vi "Transport_Receive_Command.vi"(8 "error in (no error)":errorcluster={"status"=FALSE, "code"=0, "source"="\"\""}, 10 "shutdown token":string, 11 "Transport ref":string) -> (0 "error out":errorcluster={"status"=FALSE, "code"=0, "source"="\"\""}, 2 "status ok":bool, 3 "RuntimeMessage":string)   [LabVIEW 2026]
doc: "INTENT: Consume incoming target requests. LOGIC: Read with bounded timeout; decode and validate envelope; reject malformed messages."
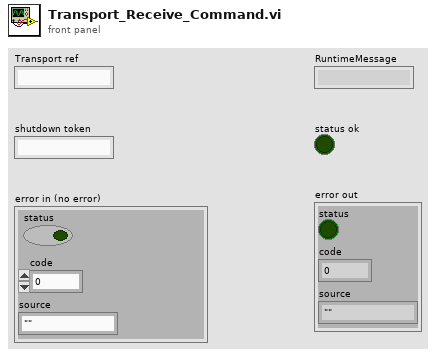
[diagram p1: front panel]
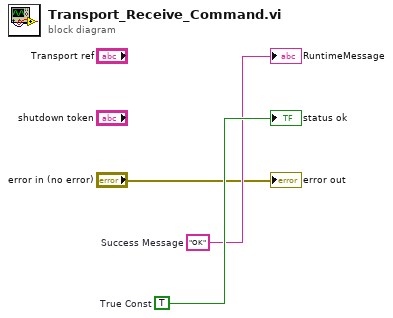
[diagram p0: block diagram]
diagram:
  w3 = TRUE  # True Const
  w2 = "OK"  # Success Message
  "RuntimeMessage" <- w2
  "status ok" <- w3
  "error out" <- "error in (no error)"
